vi "Caller.vi"(11 "error in":errorcluster) -> (2 "Count":i32, 15 "error out":errorcluster)   [LabVIEW 2026]
doc: "Issue 136 example: reads Count from an Outer typedef constant, which nests the Inner typedef."
uses:
  Outer.ctl
  Inner.ctl
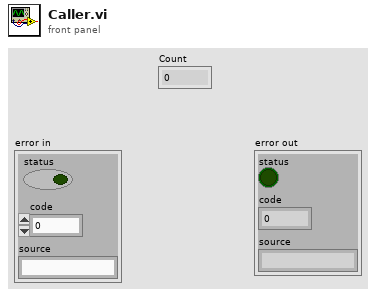
[diagram p1: front panel]
types:
  T1 = typedef "Outer.ctl" = cluster{"Inner":T2, "Count":i32}
  T2 = typedef "Inner.ctl" = cluster{"A":dbl}
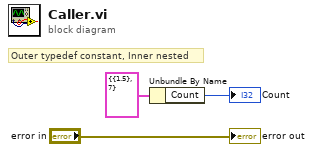
[diagram p0: block diagram]
diagram:
  # "Outer typedef constant, Inner nested"
  n1 = Unbundle By Name(T1 {"Inner"={"A"=1.5}, "Count"=7} ("Outer")) -> ("Count"=→"Count":i32)
  "error out" <- "error in"
